vi "Status Due.vi"(9 "interval (ms)":u32=1000, 10 "now (ms)":u32, 11 "last tick (ms)":u32) -> (3 "due":bool)   [LabVIEW 2021, in "CAN RW CANsub.lvclass"]
doc: "True if interval (ms) or more passed from last tick (ms) to now (ms). Correct across a rollover of the tick counter. Loop-safe: no allocation, bounded time."
uses:
  CAN RW CANsub.lvclass
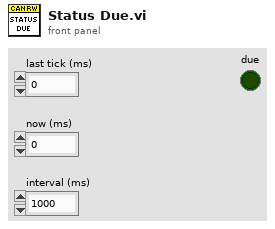
[diagram p1: front panel]
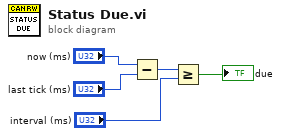
[diagram p0: block diagram]
diagram:
  n1 = Subtract(x="now (ms)", y="last tick (ms)") -> (x-y=w3:u32)
  n2 = Greater Or Equal?(x=w3, y="interval (ms)") -> (x >= y?=→"due":bool)
